vi "Low Pass Filter.vi"(6 "order":i32=2, 8 "Error In":errorcluster, 9 "Time constant":dbl=1.0, 10 "Sample rate":dbl=1.0, 11 "Data":cdb[](array[numeric])) -> (0 "Error Out":errorcluster, 3 "Data out":cdb[](array[numeric]))   [LabVIEW 2016]
uses:
  <vilib>/Analysis/3filter.llb/Filter Passband Type.ctl
  <vilib>/Analysis/3filter.llb/Butterworth Filter (CDB).vi
  <vilib>/Analysis/NI_AALBase.lvlib
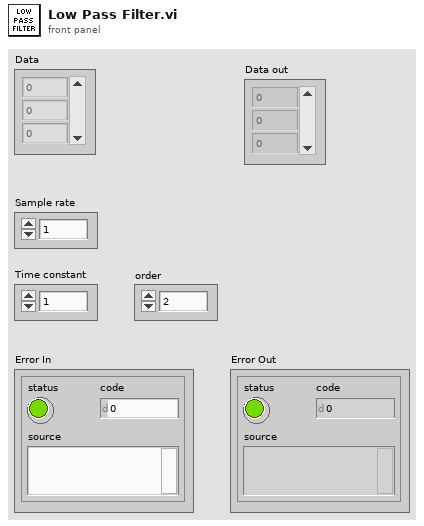
[diagram p1: front panel]
types:
  T1 = typedef "NI_AALBase.lvlib/Filter Passband Type.ctl" = enum32{"Lowpass", "Highpass", "Bandpass", "Bandstop"}
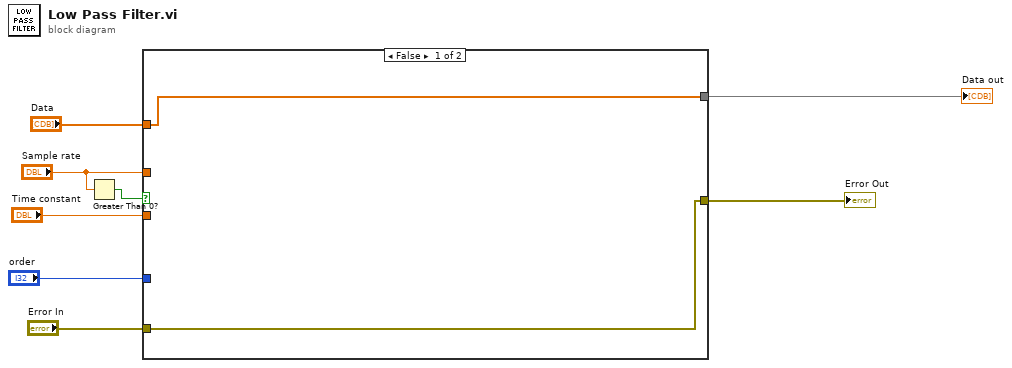
[diagram p0: block diagram]
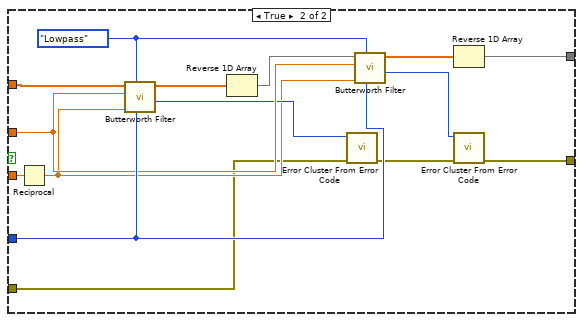
[diagram p2: hidden frame]
diagram:
  n1 = Greater Than 0?(x="Sample rate") -> (x > 0?=w2:bool)
  n2 = case shown="False" w2 {
    tunnel: "order" -> [_ w22]
    tunnel: "Data" -> [w10 w21]
    tunnel: [w10 w20] -> w6
    tunnel: "Sample rate" -> [_ w19]
    tunnel: [w9 w17] -> w5
    tunnel: "Time constant" -> [_ w14]
    tunnel: "Error In" -> [w9 w11]
    frame False {
    }
    frame True {
      w12 = Filter_Passband_Type."Lowpass" ("filter type")
      n3 = Reciprocal(x=w14) -> (1/x=w13:dbl)
      n4 = call-poly <vilib>:"Butterworth Filter.vi"("order"=w22, "filter type"=w12, "low cutoff freq: fl"=w13, "sampling freq: fs"=w19, "X"=w21) -> ("error"=w16:i32, "Filtered X"=w25:cdb[])  [unwired: 3 in]
      n5 = Reverse 1D Array(array=w25) -> (reversed array=w24:cdb[])
      n6 = call <vilib>:"Error Cluster From Error Code.vi"("error in (no error)"=w11, "error code (0)"=w16) -> ("error out"=w18:errorcluster)  [unwired: 7 in]
      n7 = call-poly <vilib>:"Butterworth Filter.vi"("order"=w22, "filter type"=w12, "low cutoff freq: fl"=w13, "sampling freq: fs"=w19, "X"=w24) -> ("error"=w15:i32, "Filtered X"=w23:cdb[])  [unwired: 3 in]
      n8 = Reverse 1D Array(array=w23) -> (reversed array=w20:cdb[])
      n9 = call <vilib>:"Error Cluster From Error Code.vi"("error in (no error)"=w18, "error code (0)"=w15) -> ("error out"=w17:errorcluster)  [unwired: 7 in]
    }
  }
  "Data out" <- w6
  "Error Out" <- w5
